vi "G-Parse-Uart_config2.vi"(8 "error in (no error)":errorcluster caption="错误输入（无错误）", 10 "配置数组":string[][](array[string])=[["串口1", "com1", "9600", "8", "0", "0", "0", "10", "10", "0"], ["串口2", "com2", "9600", "8", "0", "0", "0", "10", "10", "0"]], 11 "G-Uart-Class 输入":refnum<class "G-Uart-Class.lvclass">) -> (0 "error out":errorcluster caption="错误输出", 2 "数组":T1(array[cluster]), 3 "G-Uart-Class 输出":refnum<class "G-Uart-Class.lvclass">)   [LabVIEW 2025, in "G-Uart-Class.lvclass"]
uses:
  G-Uart-Class.lvclass
  G-Uart-Class.lvclass/G-Uart-Class.ctl
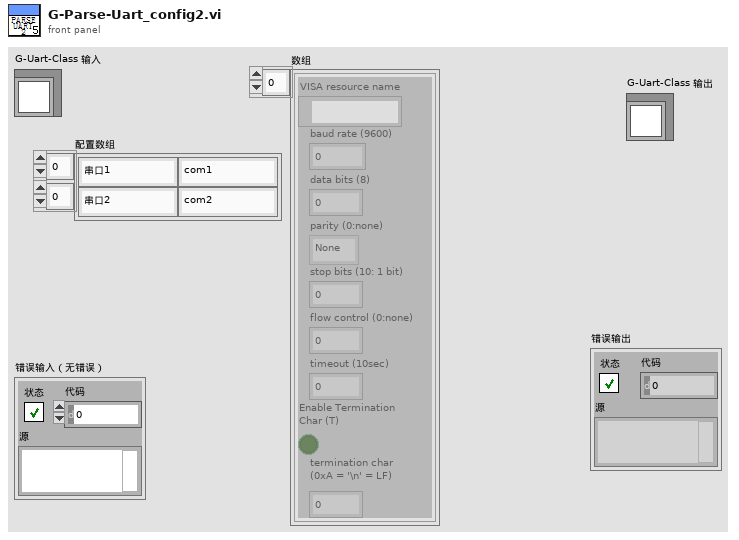
[diagram p1: front panel]
types:
  T1 = cluster{"VISA resource name":refnum<visa-resource-name>, "baud rate (9600)":u32, "data bits (8)":u16, "parity (0:none)":enum16{"None", "Odd", "Even", "Mark", "Space"}, "stop bits (10: 1 bit)":u16, "flow control (0:none)":u16, "timeout (10sec)":u32, "Enable Termination\nChar (T)":bool, "termination char\n(0xA = '\\n' = LF) ":u8}[]
  T2 = cluster{"VISA resource name":refnum<visa-resource-name>, "baud rate (9600)":u32, "data bits (8)":u16, "parity (0:none)":enum16{"None", "Odd", "Even", "Mark", "Space"}, "stop bits (10: 1 bit)":u16, "flow control (0:none)":u16, "timeout (10sec)":u32, "Enable Termination\nChar (T)":bool, "termination char\n(0xA = '\\n' = LF) ":u8}
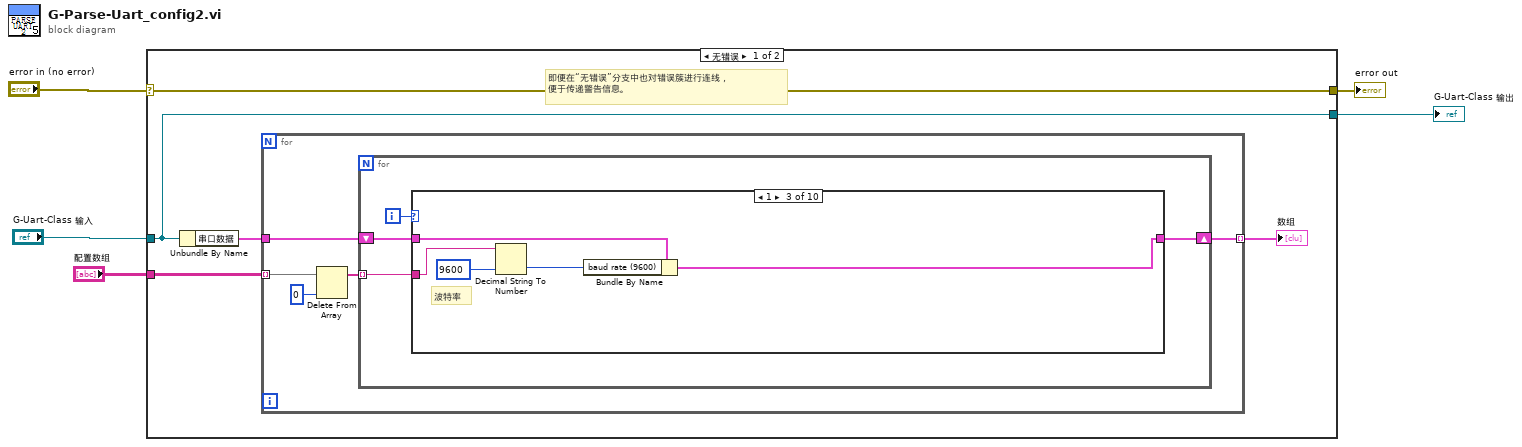
[diagram p0: block diagram]
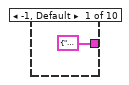
[diagram p2: hidden frame]
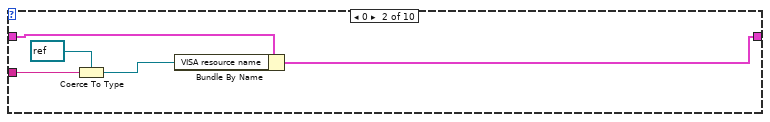
[diagram p3: hidden frame]
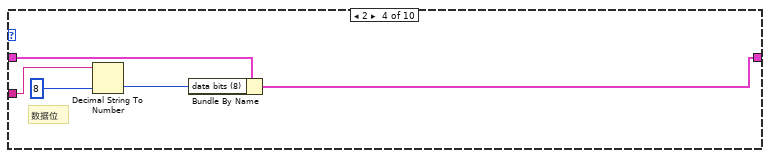
[diagram p4: hidden frame]
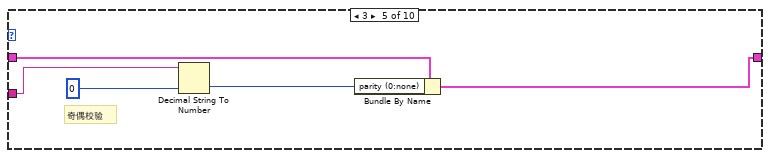
[diagram p5: hidden frame]
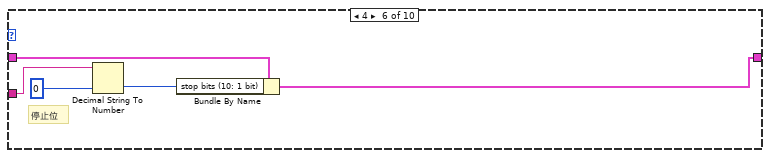
[diagram p6: hidden frame]
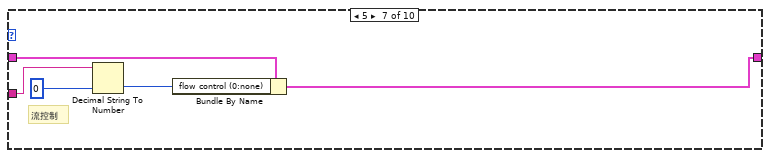
[diagram p7: hidden frame]
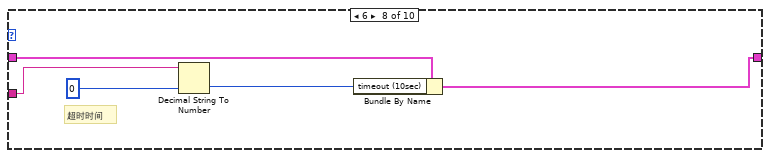
[diagram p8: hidden frame]
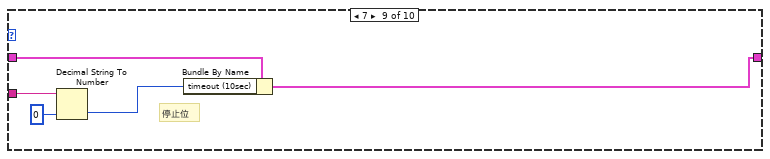
[diagram p9: hidden frame]
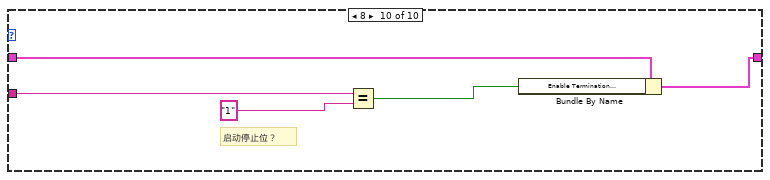
[diagram p10: hidden frame]
diagram:
  n1 = case shown="无错误" "error in (no error)" {
    selector: "error in (no error)" -> [w10 w67]
    tunnel: [w10 w67] -> w4
    tunnel: [w8 w66] -> w2
    tunnel: "G-Uart-Class 输入" -> [w8 w66]
    tunnel: "配置数组" -> [w9 _]
    frame No Error {
      # "即便在“无错误”分支中也对错误簇进行连线，\n便于传递警告信息。"
      n2 = Unbundle By Name(w8) -> ("串口数据"=w7:T2)
      n3 = for {
        tunnel: w9 -> [w14] mode=indexing
        tunnel: w7 -> [w12]
        tunnel: [w11] -> w6 mode=indexing
        n4 = Delete From Array(array=w14, index=0 ("索引")) -> (array with subset deleted=w15:string[])  [unwired: 1 in, 1 out]
        n5 = for {
          tunnel: w15 -> [w18] mode=indexing
          shift-right: [w16] -> w11
          shift-left: w12 -> [w17]
          i -> [w19]
          n6 = case shown="1" w19 {
            tunnel: w18 -> [_ w24 w30 w35 w40 w45 w50 w55 w60 w63]
            tunnel: [T2 {"VISA resource name"="", "baud rate (9600)"=9600, "data bits (8)"=8, "parity (0:none)"=enum."None", "stop bits (10: 1 bit)"=10, "flow control (0:none)"=0, "timeout (10sec)"=10000, "Enable Termination\nChar (T)"=TRUE, "termination char\n(0xA = '\\n' = LF) "=10} ("簇") w22 w28 w33 w38 w43 w48 w53 w58 w65] -> w16
            tunnel: w17 -> [_ w21 w27 w32 w37 w42 w47 w52 w57 w64]
            frame -1, Default {
            }
            frame 0 {
              n7 = Coerce To Type(0:w24, 1:refnum<visa-resource-name> refnum ("VISA resource name")) -> (2:w23:refnum<visa-resource-name>)
              n8 = Bundle By Name(cluster=w21, "VISA resource name"=w23) -> (w22:T2)
            }
            frame 1 {
              # "波特率"
              n9 = Decimal String To Number(string=w30, default (0L)=u64 9600 ("baud rate (9600)")) -> (number=w26:u64)  [unwired: 1 in, 1 out]
              n10 = Bundle By Name(cluster=w27, "baud rate (9600)"=w26) -> (w28:T2)
            }
            frame 2 {
              # "数据位"
              n11 = Decimal String To Number(string=w35, default (0L)=8 ("baud rate (9600)")) -> (number=w31:i32)  [unwired: 1 in, 1 out]
              n12 = Bundle By Name(cluster=w32, "data bits (8)"=w31) -> (w33:T2)
            }
            frame 3 {
              # "奇偶校验"
              n13 = Decimal String To Number(string=w40, default (0L)=0 ("baud rate (9600)")) -> (number=w36:i32)  [unwired: 1 in, 1 out]
              n14 = Bundle By Name(cluster=w37, "parity (0:none)"=w36) -> (w38:T2)
            }
            frame 4 {
              # "停止位"
              n15 = Decimal String To Number(string=w45, default (0L)=0 ("baud rate (9600)")) -> (number=w41:i32)  [unwired: 1 in, 1 out]
              n16 = Bundle By Name(cluster=w42, "stop bits (10: 1 bit)"=w41) -> (w43:T2)
            }
            frame 5 {
              # "流控制"
              n17 = Decimal String To Number(string=w50, default (0L)=0 ("baud rate (9600)")) -> (number=w46:i32)  [unwired: 1 in, 1 out]
              n18 = Bundle By Name(cluster=w47, "flow control (0:none)"=w46) -> (w48:T2)
            }
            frame 6 {
              # "超时时间"
              n19 = Decimal String To Number(string=w55, default (0L)=0 ("baud rate (9600)")) -> (number=w51:i32)  [unwired: 1 in, 1 out]
              n20 = Bundle By Name(cluster=w52, "timeout (10sec)"=w51) -> (w53:T2)
            }
            frame 7 {
              # "停止位"
              n21 = Decimal String To Number(string=w60, default (0L)=0 ("baud rate (9600)")) -> (number=w56:i32)  [unwired: 1 in, 1 out]
              n22 = Bundle By Name(cluster=w57, "timeout (10sec)"=w56) -> (w58:T2)
            }
            frame 8 {
              # "启动停止位？"
              n23 = Equal?(x=w63, y="1") -> (x = y?=w61:bool)
              n24 = Bundle By Name(cluster=w64, "Enable Termination\nChar (T)"=w61) -> (w65:T2)
            }
          }
        }
      }
      "数组" <- w6
    }
    frame Error {
    }
  }
  "error out" <- w4
  "G-Uart-Class 输出" <- w2
